vi "Status_Test.vi"() -> ()   [LabVIEW 2026]
panel:
  out "ADC Raw":dbl
  in  "stop":bool
  out "Waveform Chart":dbl(graph)
  out "Received JSON":string
  in  "port":dbl
  in  "pi_IP":string
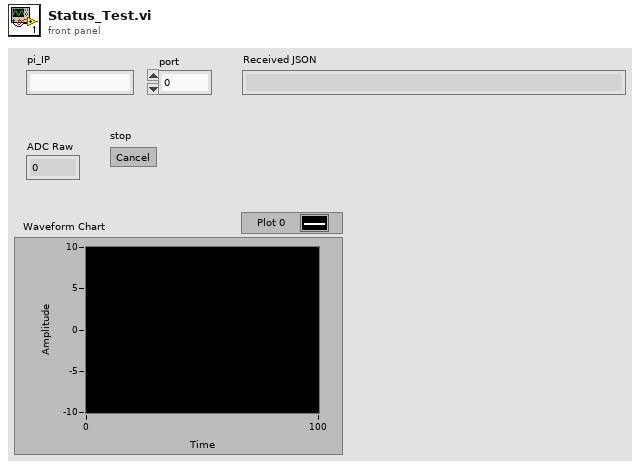
[diagram p1: front panel]
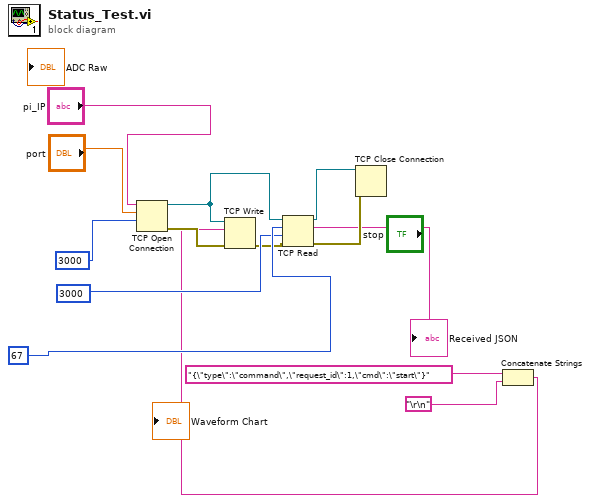
[diagram p0: block diagram]
diagram:
  n1 = TCP Open Connection(address="pi_IP", remote port or service name="port", timeout ms (60000)=3000) -> (connection ID=w9:refnum<k5>, error out=w7:errorcluster)  [unwired: 2 in]
  n2 = Concatenate Strings "Concatenate Strings"("{\"type\":\"command\",\"request_id\":1,\"cmd\":\"start\"}", "\r\n") -> (w1:string)
  n3 = TCP Write(connection ID=w9, data in=w1, error in (no error)=w7) -> (error out=w6:errorcluster)  [unwired: 1 in, 2 out]
  n4 = TCP Read(connection ID=w9, bytes to read=67, error in (no error)=w6, 9:3000) -> (connection ID out=w8:refnum<k5>, data out=→"Received JSON":string, error out=w5:errorcluster)  [unwired: 1 in]
  n5 = TCP Close Connection(connection ID=w8, error in (no error)=w5) -> ()  [unwired: 1 in, 2 out]
